vi "lab1_cw4_test.vi"() -> ()   [LabVIEW 2025]
panel:
  in  "D":i32
  in  "M":i32
  in  "milliseconds to wait":u32
  out "Waveform Chart":dbl(graph)
  in  "N":i32
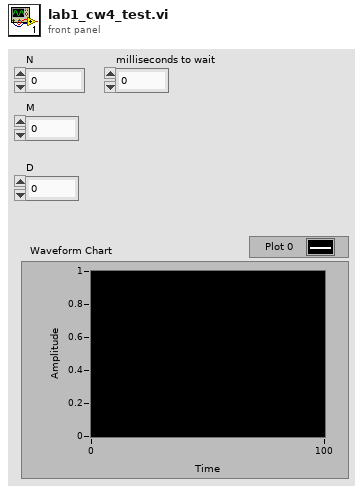
[diagram p1: front panel]
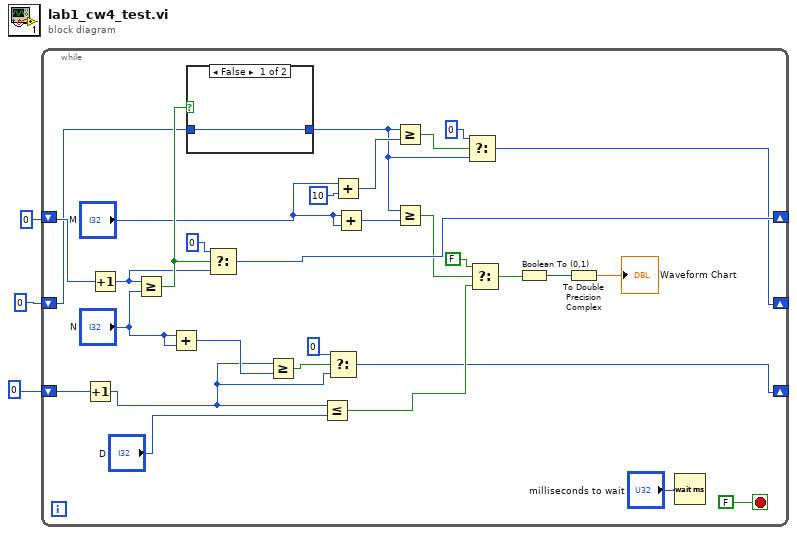
[diagram p0: block diagram]
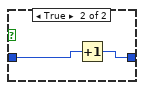
[diagram p2: hidden frame]
diagram:
  n1 = while {
    shift-right: [w31] -> _
    shift-left: 0 -> [w33]
    shift-right: [w16] -> _
    shift-left: 0 -> [w23]
    shift-right: [w7] -> _
    shift-left: 0 -> [w12]
    stop <- FALSE stop-if-true
    n2 = Increment(x=w12) -> (x+1=w8:i32)
    n3 = Increment(x=w33) -> (x+1=w14:i32)
    n4 = Greater Or Equal?(x=w14, y="N") -> (x >= y?=w24:bool)
    n5 = Add(x="N", y="N") -> (x+y=w10:i32)
    n6 = case shown="False" w24 {
      tunnel: w23 -> [w34 w35]
      tunnel: [w34 w36] -> w18
      frame False {
      }
      frame True {
        n7 = Increment(x=w35) -> (x+1=w36:i32)
      }
    }
    n8 = Select(t=0, s=w24, f=w14) -> (s? t:f=w31:i32)
    n9 = Greater Or Equal?(x=w8, y=w10) -> (x >= y?=w9:bool)
    n10 = Less Or Equal?(x=w8, y="D") -> (x <= y?=w15:bool)
    n11 = Select(t=0, s=w9, f=w8) -> (s? t:f=w7:i32)
    n12 = Add(x="M", y=10) -> (x+y=w20:i32)
    n13 = Add(x="M", y="M") -> (x+y=w4:i32)
    n14 = Greater Or Equal?(x=w18, y=w20) -> (x >= y?=w19:bool)
    n15 = Greater Or Equal?(x=w18, y=w4) -> (x >= y?=w26:bool)
    n16 = Select(t=0, s=w19, f=w18) -> (s? t:f=w16:i32)
    n17 = Select(t=FALSE, s=w26, f=w15) -> (s? t:f=w22:bool)
    n18 = Boolean To (0,1)(Boolean=w22) -> (0, 1=w29:i16)
    n19 = To Double Precision Complex(1:w29) -> (0:→"Waveform Chart":cdb)
    n20 = Wait (ms)(milliseconds to wait="milliseconds to wait") -> ()  [unwired: 1 out]
  }
